vi "Shutdown.vi"(7 "Refnum out 3":refnum<k20>, 8 "error in (no error)":errorcluster, 9 "Refnum in":refnum<k21>, 10 "rt fifo ref in":refnum<k33>, 11 "Refnum in":refnum<k21>) -> (0 "error out":errorcluster)   [LabVIEW 2025]
uses:
  <vilib>/rvi/interface/nirviCloseFPGA/nirviCloseFPGA.xnode
  <vilib>/FPGAPlugInAG/Dynamic/niLvFpga_Close_Dynamic.vi
  <vilib>/dex/Flush And Wait Empty Condition.ctl
  Command.ctl
  vi/thresholds.ctl
  RT_Cmd.ctl
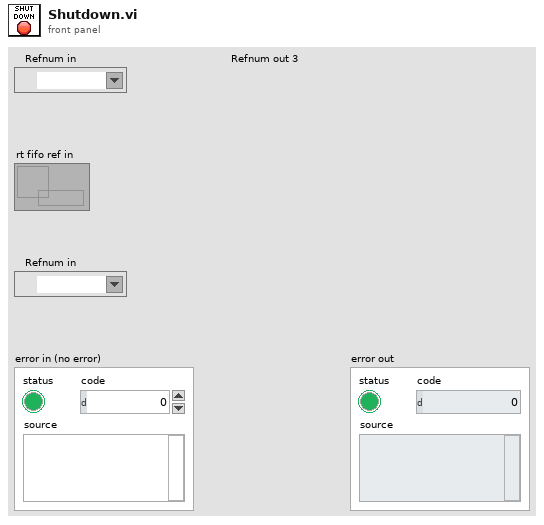
[diagram p1: front panel]
types:
  T1 = typedef "Flush And Wait Empty Condition.ctl" = u8
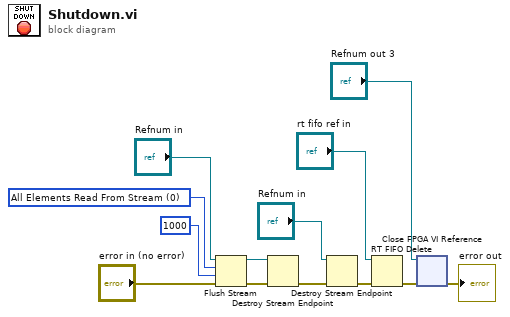
[diagram p0: block diagram]
diagram:
  w3 = T1 0 items=["All Elements Read From Stream", "All Elements Available for Reading"] ("wait condition")
  n1 = Flush Stream(8:"error in (no error)", 9:1000 ("timeout in ms (-1)"), 10:w3, 11:"Refnum in") -> (0:w2:errorcluster, 3:w10:refnum<k21>)  [unwired: 1 out]
  n2 = Destroy Stream Endpoint(8:w2, 11:w10) -> (0:w11:errorcluster)
  n3 = Destroy Stream Endpoint(8:w11, 11:"Refnum in") -> (0:w12:errorcluster)
  n4 = RT FIFO Delete(0:"rt fifo ref in", 3:w12) -> (11:w4:errorcluster)  [unwired: 1 in]
  n5 = xnode "Close FPGA VI Reference"("FPGA VI Reference In"="Refnum out 3", "error in"=w4) -> ("error out"=→"error out":errorcluster)
